vi "PicoScope2000aGetTimebase2.vi"(4 "Number of Samples":u32, 6 "Memory Segment":u32, 7 "Acquisition Settings":T1 {"postTriggerSamples" format="%_6p"; "preTriggerSamples" format="%_6p"}, 8 "error in (no error)":errorcluster, 11 "handle in":i16) -> (0 "error out":errorcluster, 3 "handle out":i16, 5 "Properties Panel":T2 {"Max Total Capture Time Available (sec)" format="%.3p"; "Sample Frequency" format="%.3p"; "Sample Internal" format="%.3p"; "Max Samples Available" format="%.3p"; "Total Capture Time (sec)" format="%.3p"})   [LabVIEW 2009]
uses:
  ps2000a.dll
  shared/Acquisition Settings.ctl
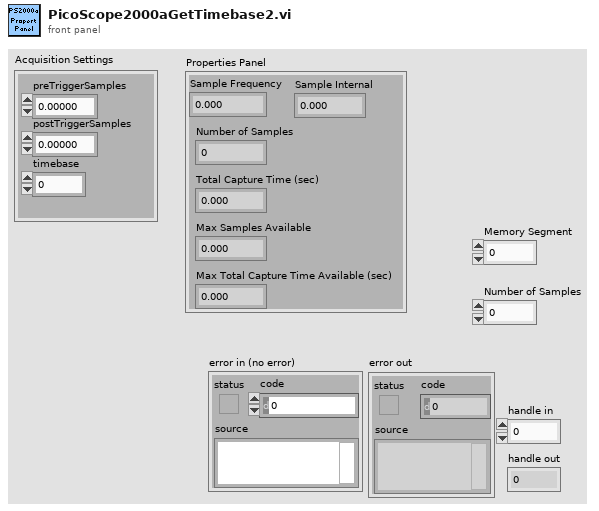
[diagram p1: front panel]
types:
  T1 = typedef "Acquisition Settings.ctl" = cluster{"preTriggerSamples":u64, "postTriggerSamples":u64, "timebase":u32}
  T2 = cluster{"Sample Frequency":sgl, "Sample Internal":sgl, "Max Samples Available":i32, "Number of Samples":u32, "Total Capture Time (sec) ":sgl, "Max Total Capture Time Available (sec)":sgl}
  T3 = cluster{sgl, sgl, "maxSamples":i32, "Number of Samples":u32, sgl, sgl}
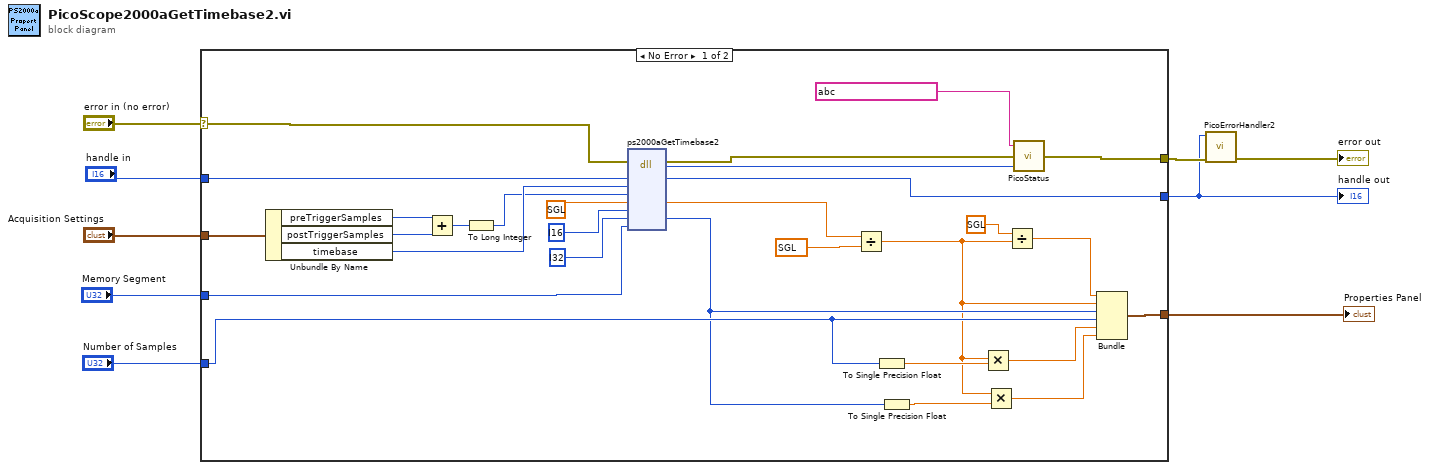
[diagram p0: block diagram]
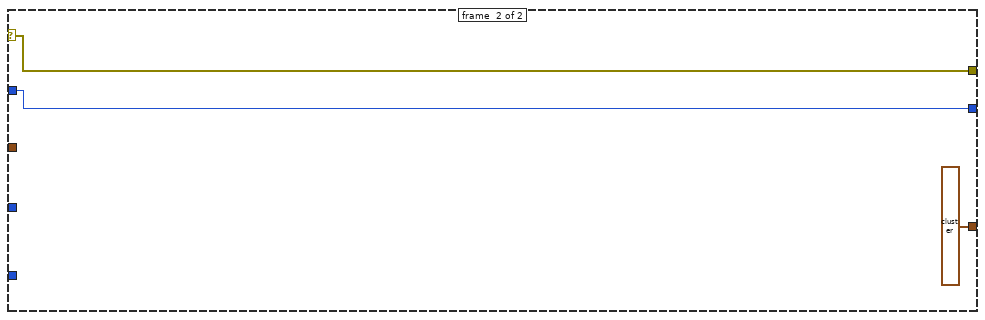
[diagram p2: hidden frame]
diagram:
  n1 = case shown="No Error" "error in (no error)" {
    selector: "error in (no error)" -> [w10 w41]
    tunnel: [w30 w41] -> w4
    tunnel: [w29 w40] -> w2
    tunnel: "Memory Segment" -> [w11 _]
    tunnel: "Number of Samples" -> [w24 _]
    tunnel: "handle in" -> [w28 w40]
    tunnel: "Acquisition Settings" -> [w27 _]
    tunnel: [w20 T3 ?] -> w5
    frame #0 {
      n2 = Unbundle By Name(w27) -> ("preTriggerSamples"=w33:u64, "postTriggerSamples"=w34:u64, "timebase"=w35:u32)
      n3 = Add(x=w33, y=w34) -> (x+y=w13:u64)
      n4 = To Long Integer(number=w13) -> (32bit integer=w12:i32)
      n5 = dll-call lib="ps2000a.dll" fn="ps2000aGetTimebase2"(error in=w10, "handle"=w28, "timebase"=w35, "noSamples"=w12, "timeIntervalNanoseconds"=sgl ?, "oversample"=i16 ?, "maxSamples"=i32 ?, "segmentIndex"=w11) -> (error out=w36:errorcluster, "PICO_STATUS"=w31:u32, "handle"=w29:i16, "timeIntervalNanoseconds"=w37:sgl, "maxSamples"=w22:i32)  [unwired: 6 in, 1 out]
      n6 = Divide(x=w37, y=sgl ?) -> (x/y=w15:sgl)
      n7 = To Single Precision Float(number=w24) -> (single precision float=w26:sgl)
      n8 = To Single Precision Float(number=w22) -> (single precision float=w23:sgl)
      n9 = Multiply(x=w15, y=w26) -> (x*y=w25:sgl)
      n10 = Multiply(x=w15, y=w23) -> (x*y=w21:sgl)
      n11 = Divide(x=sgl ?, y=w15) -> (x/y=w16:sgl)
      n12 = call "PicoStatus.vi"("PICO STATUS"=w31, "error in"=w36, "source"=string ?) -> ("error out"=w30:errorcluster)
      n13 = Bundle(w16, w15, "maxSamples"=w22, "Number of Samples"=w24, w25, w21) -> (w20:T3)  [unwired: 1 in]
    }
    frame #1 {
    }
  }
  "handle out" <- w2
  "Properties Panel" <- w5
  n14 = call "PicoErrorHandler2.vi"("error in (no error)"=w4, "handle In"=w2) -> ("error out"=→"error out":errorcluster)  [unwired: 9 in]
